vi "Stop.vi"(8 "error in (no error)":errorcluster, 11 "ArrayManager in":refnum<class "ArrayManager.lvclass">) -> (0 "error out":errorcluster, 3 "ArrayManager out":refnum<class "ArrayManager.lvclass">)   [LabVIEW 2020, in "OOPanel.lvlib" / "ArrayManager.lvclass"]
uses:
  ArrayManager.lvclass
  ArrayManager.lvclass/ArrayManager.ctl
panel:
  out "call chain":string[](array[string])
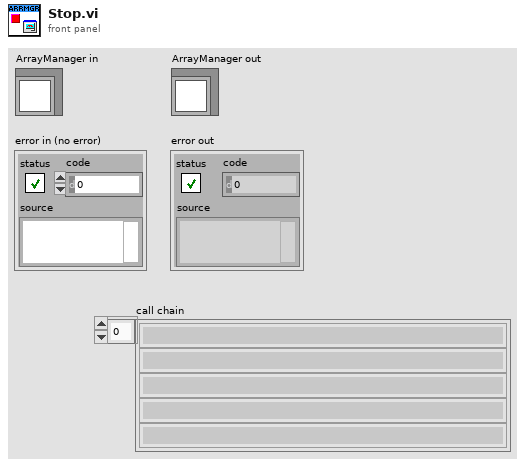
[diagram p1: front panel]
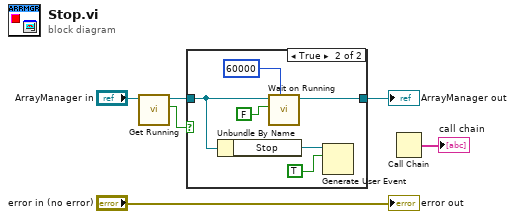
[diagram p0: block diagram]
diagram:
  n1 = call "Get Running.vi"("ArrayManager in"="ArrayManager in") -> ("Running"=w2:bool, "ArrayManager out"=w4:refnum<class "ArrayManager.lvclass">)  [unwired: 8 in, 1 out]
  n2 = case shown="True" w2 {
    tunnel: w4 -> [w7 w9]
    tunnel: [w7 w11] -> w3
    frame False {
    }
    frame True {
      n3 = Unbundle By Name(w9) -> ("Stop"=w13:refnum<user-event>)
      n4 = call "Wait on Running.vi"("Timeout (10000ms)"=60000, "Value"=FALSE, "ArrayManager in"=w9) -> ("ArrayManager out"=w11:refnum<class "ArrayManager.lvclass">)  [unwired: 7 in, 1 out]
      n5 = Generate User Event(user event=w13, event data cluster=TRUE ("event data")) -> ()  [unwired: 2 in, 2 out]
    }
  }
  "ArrayManager out" <- w3
  n6 = Call Chain() -> (call chain=→"call chain":string[])
  "error out" <- "error in (no error)"
